vi "Voir alertes.vi"() -> ()   [LabVIEW 2022 SP3]
uses:
  Enum/Enum 8.ctl
  Variables globales/Variable glob alertes ecart temperatures.vi
  Variables globales/Variable glob alertes pressions.vi
  Variables globales/Variable glob alertes min-max temperatures.vi
  Variables globales/Variable glob mails.vi
  Variables globales/Variable glob alertes Compteurs.vi
  Variables globales/Variable glob alertes Keller.vi
panel:
  out "référence en sortie":refnum<vi>
  in  "stop":bool
  in  "Commande onglets":T1(tab)
  out "min-max temp":T2(array[cluster]) {"alerte min (°C) :" format="%.2f"; "alerte max (°C) :" format="%.2f"}
  out "écarts températures":T3(array[cluster]) {"alerte écart (°C) :" format="%.2f"}
  out "Pressions":T4(array[cluster]) {"alerte pression (mbar) :" format="%.2e"}
  out "Keller":T5(array[cluster]) {"alerte keller (mbar) :" format="%.2g"}
  out "Copmteurs":T6(array[cluster]) {"alerte débit compteurs (m3/h) :" format="%.2g"}
  out "Liste mails envoi alertes":string[](array[string])
  # "capteurs surveillés :"
  # "Ce logiciel et les informations qu'il contient, sont la propriété de l’IAS \net ne peuvent être diffusés sans l’autorisation de la Station d’étalonnage"
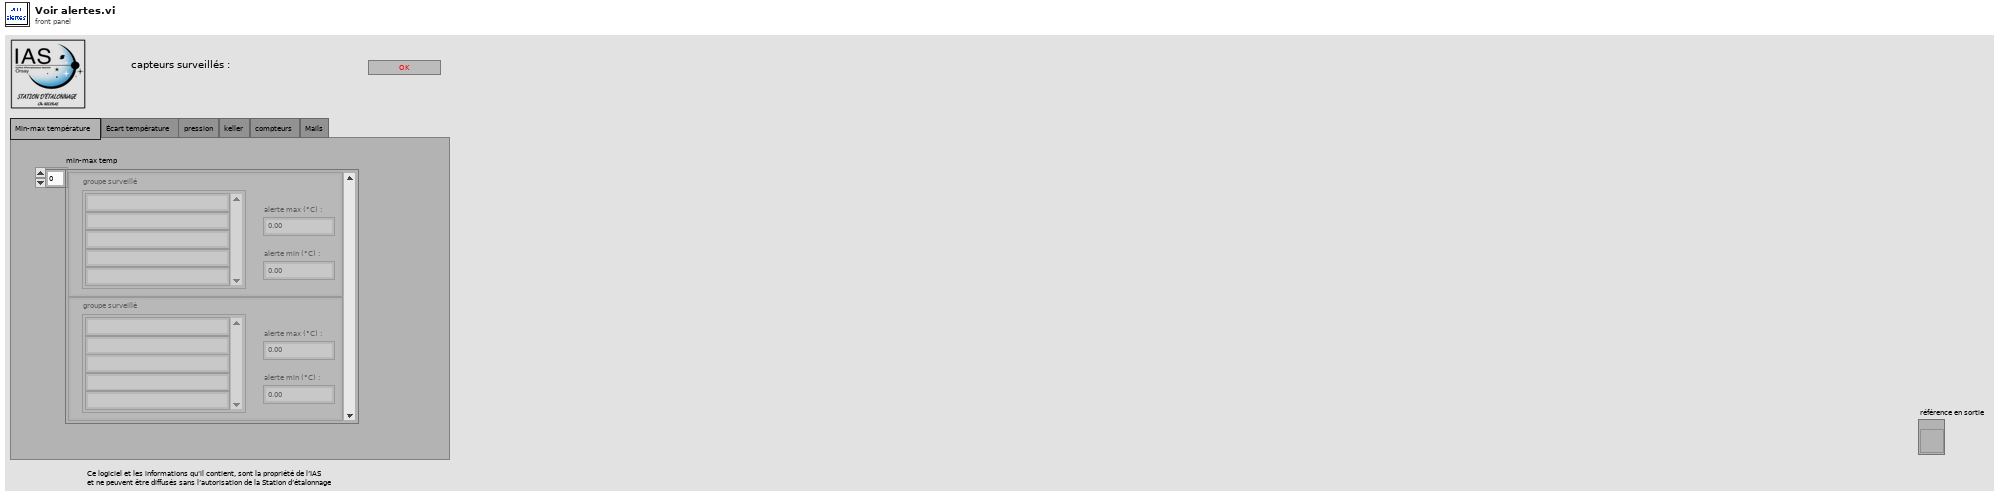
[diagram p1: front panel]
types:
  T1 = enum32{"Min-max température", "Écart température", "pression", "keller", "compteurs", "Mails"}
  T2 = cluster{"groupe surveillé":string[], "alerte max (°C) :":dbl, "alerte min (°C) :":dbl}[]
  T3 = cluster{"capteurs temp surveillés":string[], "alerte écart (°C) :":dbl, ">?":bool}[]
  T4 = cluster{"capteurs pression surveillés":string[], "alerte pression (mbar) :":dbl}[]
  T5 = cluster{"capteurs keller surveillés":string[], "alerte keller (mbar) :":dbl}[]
  T6 = cluster{"compteurs débit surveillés":string[], "alerte débit compteurs (m3/h) :":dbl}[]
  T7 = typedef "Enum 8.ctl" = enum16{"init", "variables", "variables 2", "onglets", "attente", "fin"}
  T8 = enum32{"Invalid", "Standard", "Closed", "Hidden", "Minimized", "Maximized"}
  T9 = cluster{"Alerte temp min/max":bool, "température max":dbl, "température min":dbl, "Défaut min/max temp":bool, "Indices à controler":i16[], "N°":u16}[]
  T10 = cluster{"Indices a controler":i16[], "Defaut":bool, "ecart temp":dbl, "Alerte":bool, ">?":bool, "N°":u16}[]
  T11 = cluster{"Alerte":bool, "valeur ":dbl, "Défaut":bool, "Indices controler":i16[], "N°":u16}[]
  T12 = cluster{"capteurs temp surveillés":string[], "alerte écart (°C) :":dbl, ">?":bool}
  T13 = cluster{"capteurs pression surveillés":string[], "alerte pression (mbar) :":dbl}
  T14 = cluster{"groupe surveillé":string[], "alerte max (°C) :":dbl, "alerte min (°C) :":dbl}
  T15 = cluster{"Alerte":bool, "valeur alerte":dbl, "Défaut":bool, "Indices à controler":i16[], "N°":u16}[]
  T16 = cluster{"Alerte Keller":bool, "valeur alerte Keller":dbl, "Défaut Keller":bool, "Indices Keller à controler":i16[], "N°":u16}[]
  T17 = cluster{"compteurs débit surveillés":string[], "alerte débit compteurs (m3/h) :":dbl}
  T18 = cluster{"capteurs keller surveillés":string[], "alerte keller (mbar) :":dbl}
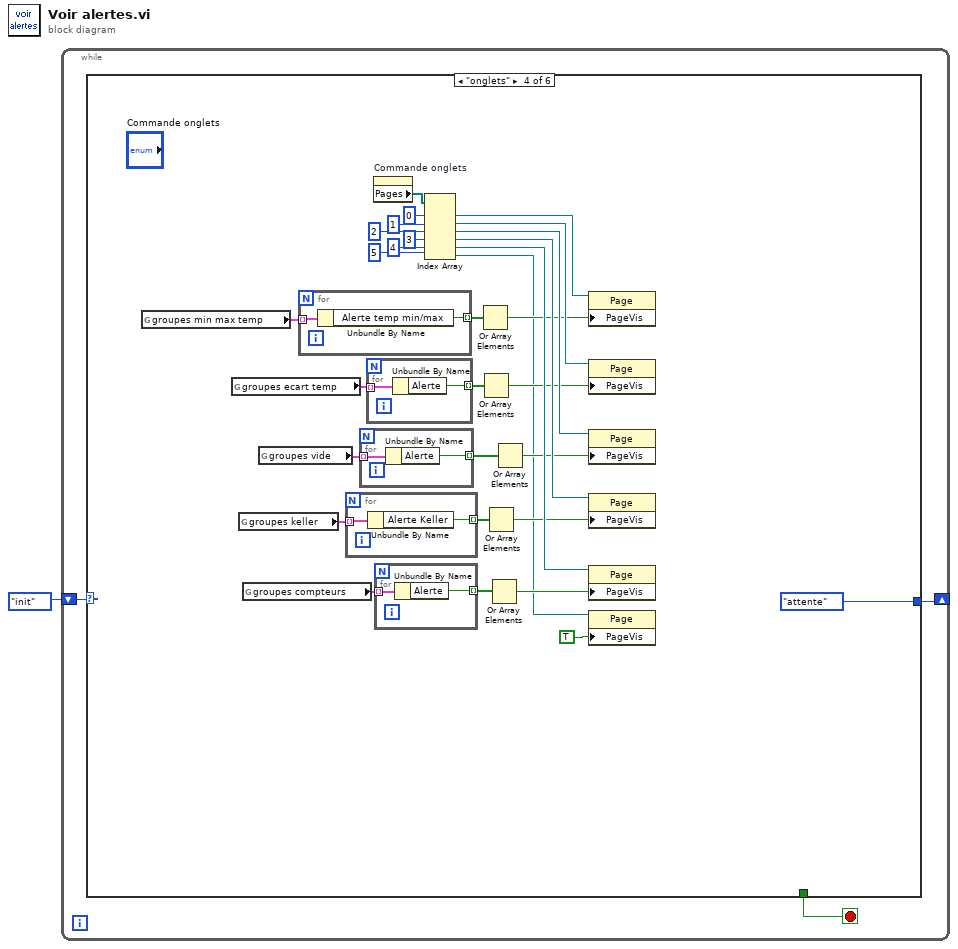
[diagram p0: block diagram]
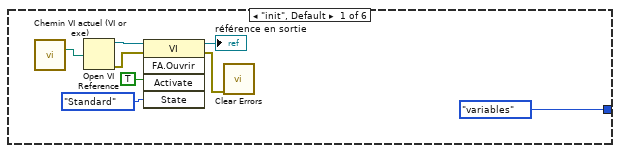
[diagram p2: hidden frame]
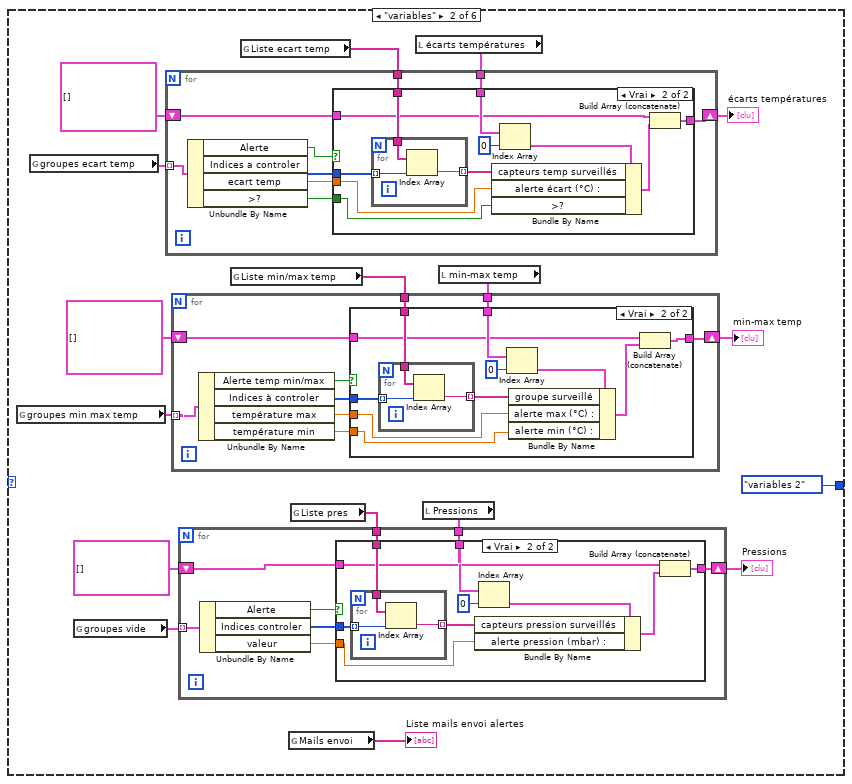
[diagram p3: hidden frame]
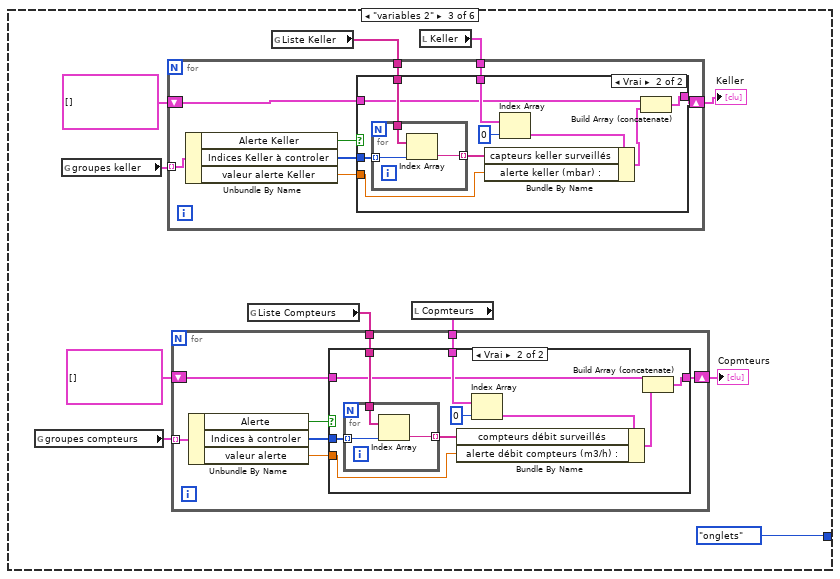
[diagram p7: hidden frame]
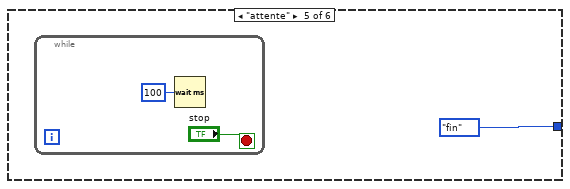
[diagram p10: hidden frame]
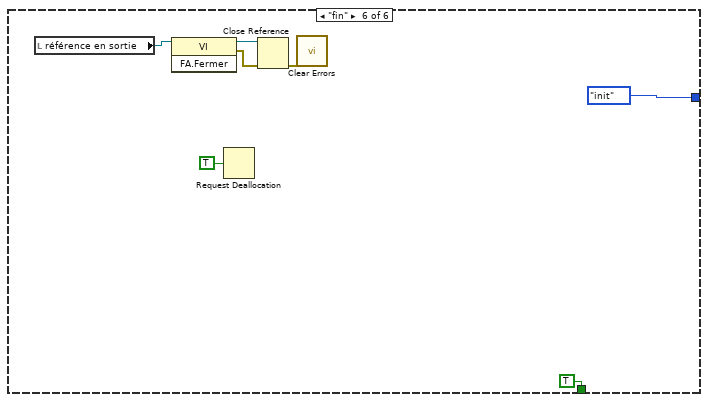
[diagram p11: hidden frame]
diagram:
  n1 = while {
    shift-right: [w3] -> _
    shift-left: Enum_8."init" ("Énum") -> [w4]
    stop <- w2 stop-if-true
    n2 = case shown="\"onglets\"" w4 {
      tunnel: [Enum_8."variables" ("Énum") Enum_8."variables 2" ("Énum") Enum_8."onglets" ("Énum") Enum_8."attente" ("Énum") Enum_8."fin" ("Énum") Enum_8."init" ("Énum")] -> w3
      tunnel: [_ _ _ _ _ TRUE] -> w2
      frame "init", Default {
        n3 = call "Chemin VI actuel (VI or exe).vi"() -> ("Full Path to VI or executable"=w5:path)  [unwired: 14 in, 1 out]
        n4 = Open VI Reference(vi path=w5) -> (vi reference=w9:refnum<vi>, error out=w11:errorcluster)  [unwired: 5 in]
        n5 = invoke class="VI" method="FA.Ouvrir"(reference=w9, error in=w11, "Activate"=TRUE ("Activer ?"), "State"=T8."Standard" ("État")) -> (reference out=→"référence en sortie":refnum<vi>, error out=w12:errorcluster)  [unwired: 1 in, 3 out]
        n6 = call <vilib>:"Clear Errors.vi"("error in (no error)"=w12) -> ()  [unwired: 5 in, 2 out]
      }
      frame "variables" {
        n7 = global read "Variable glob alertes min-max temperatures.vi" "groupes min max temp"() -> (w24:T9)
        n8 = global read "Variable glob alertes ecart temperatures.vi" "groupes ecart temp"() -> (w28:T10)
        n9 = global read "Variable glob alertes pressions.vi" "groupes vide"() -> (w21:T11)
        n10 = global read "Variable glob alertes min-max temperatures.vi" "Liste min/max temp"() -> (w23:string[])
        n11 = global read "Variable glob alertes ecart temperatures.vi" "Liste ecart temp"() -> (w27:string[])
        n12 = global read "Variable glob mails.vi" "Mails envoi"() -> (→"Liste mails envoi alertes":string[])
        n13 = global read "Variable glob alertes pressions.vi" "Liste pres"() -> (w22:string[])
        n14 = local read "écarts températures"() -> (w26:T3)
        n15 = for {
          tunnel: w28 -> [w84] mode=indexing
          tunnel: w27 -> [w82]
          tunnel: w26 -> [w81]
          shift-right: [w76] -> w20
          shift-left: T3 [] -> [w77]
          n16 = Unbundle By Name(w84) -> ("Alerte"=w79:bool, "Indices a controler"=w83:i16[], "ecart temp"=w80:dbl, ">?"=w78:bool)
          n17 = case shown="Vrai" w79 {
            tunnel: w83 -> [_ w96]
            tunnel: w82 -> [_ w95]
            tunnel: w81 -> [_ w94]
            tunnel: w80 -> [_ w90]
            tunnel: w78 -> [_ w89]
            tunnel: w77 -> [w85 w87]
            tunnel: [w85 w86] -> w76
            frame False {
            }
            frame True {
              n18 = for {
                tunnel: w96 -> [w98] mode=indexing
                tunnel: w95 -> [w99]
                tunnel: [w97] -> w91 mode=indexing
                n19 = Index Array(array=w99, index=w98) -> (element=w97:string)
              }
              n20 = Index Array(array=w94, index=0 ("indice")) -> (element=w92:T12)
              n21 = Bundle By Name(cluster=w92, "capteurs temp surveillés"=w91, "alerte écart (°C) :"=w90, ">?"=w89) -> (w88:T12)
              n22 = Build Array (concatenate)(w87, w88) -> (w86:T3)
            }
          }
        }
        "écarts températures" <- w20
        n23 = local read "Pressions"() -> (w16:T4)
        n24 = for {
          tunnel: w21 -> [w37] mode=indexing
          tunnel: w22 -> [w35]
          tunnel: w16 -> [w34]
          shift-right: [w30] -> w15
          shift-left: T4 [] -> [w31]
          n25 = Unbundle By Name(w37) -> ("Alerte"=w32:bool, "Indices controler"=w36:i16[], "valeur"=w33:dbl)
          n26 = case shown="Vrai" w32 {
            tunnel: w36 -> [_ w48]
            tunnel: w35 -> [_ w47]
            tunnel: w34 -> [_ w46]
            tunnel: w33 -> [_ w42]
            tunnel: w31 -> [w38 w40]
            tunnel: [w38 w39] -> w30
            frame False {
            }
            frame True {
              n27 = for {
                tunnel: w48 -> [w50] mode=indexing
                tunnel: w47 -> [w51]
                tunnel: [w49] -> w43 mode=indexing
                n28 = Index Array(array=w51, index=w50) -> (element=w49:string)
              }
              n29 = Index Array(array=w46, index=0 ("indice")) -> (element=w44:T13)
              n30 = Bundle By Name(cluster=w44, "capteurs pression surveillés"=w43, "alerte pression (mbar) :"=w42) -> (w41:T13)
              n31 = Build Array (concatenate)(w40, w41) -> (w39:T4)
            }
          }
        }
        "Pressions" <- w15
        n32 = local read "min-max temp"() -> (w25:T2)
        n33 = for {
          tunnel: w24 -> [w60] mode=indexing
          tunnel: w23 -> [w58]
          tunnel: w25 -> [w57]
          shift-right: [w52] -> w17
          shift-left: T2 [] -> [w53]
          n34 = Unbundle By Name(w60) -> ("Alerte temp min/max"=w54:bool, "Indices à controler"=w59:i16[], "température max"=w56:dbl, "température min"=w55:dbl)
          n35 = case shown="Vrai" w54 {
            tunnel: w59 -> [_ w72]
            tunnel: w58 -> [_ w71]
            tunnel: w57 -> [_ w70]
            tunnel: w56 -> [_ w66]
            tunnel: w55 -> [_ w65]
            tunnel: w53 -> [w61 w63]
            tunnel: [w61 w62] -> w52
            frame False {
            }
            frame True {
              n36 = for {
                tunnel: w72 -> [w74] mode=indexing
                tunnel: w71 -> [w75]
                tunnel: [w73] -> w67 mode=indexing
                n37 = Index Array(array=w75, index=w74) -> (element=w73:string)
              }
              n38 = Index Array(array=w70, index=0 ("indice")) -> (element=w68:T14)
              n39 = Bundle By Name(cluster=w68, "groupe surveillé"=w67, "alerte max (°C) :"=w66, "alerte min (°C) :"=w65) -> (w64:T14)
              n40 = Build Array (concatenate)(w63, w64) -> (w62:T2)
            }
          }
        }
        "min-max temp" <- w17
      }
      frame "variables 2" {
        n41 = global read "Variable glob alertes Compteurs.vi" "groupes compteurs"() -> (w103:T15)
        n42 = global read "Variable glob alertes Keller.vi" "groupes keller"() -> (w105:T16)
        n43 = global read "Variable glob alertes Compteurs.vi" "Liste Compteurs"() -> (w104:string[])
        n44 = global read "Variable glob alertes Keller.vi" "Liste Keller"() -> (w107:string[])
        n45 = local read "Copmteurs"() -> (w102:T6)
        n46 = for {
          tunnel: w103 -> [w118] mode=indexing
          tunnel: w104 -> [w116]
          tunnel: w102 -> [w115]
          shift-right: [w111] -> w109
          shift-left: T6 [] -> [w112]
          n47 = Unbundle By Name(w118) -> ("Alerte"=w113:bool, "Indices à controler"=w117:i16[], "valeur alerte"=w114:dbl)
          n48 = case shown="Vrai" w113 {
            tunnel: w117 -> [_ w129]
            tunnel: w116 -> [_ w128]
            tunnel: w115 -> [_ w127]
            tunnel: w114 -> [_ w123]
            tunnel: w112 -> [w119 w121]
            tunnel: [w119 w120] -> w111
            frame False {
            }
            frame True {
              n49 = for {
                tunnel: w129 -> [w131] mode=indexing
                tunnel: w128 -> [w132]
                tunnel: [w130] -> w124 mode=indexing
                n50 = Index Array(array=w132, index=w131) -> (element=w130:string)
              }
              n51 = Index Array(array=w127, index=0 ("indice")) -> (element=w125:T17)
              n52 = Bundle By Name(cluster=w125, "compteurs débit surveillés"=w124, "alerte débit compteurs (m3/h) :"=w123) -> (w122:T17)
              n53 = Build Array (concatenate)(w121, w122) -> (w120:T6)
            }
          }
        }
        "Copmteurs" <- w109
        n54 = local read "Keller"() -> (w106:T5)
        n55 = for {
          tunnel: w105 -> [w140] mode=indexing
          tunnel: w107 -> [w138]
          tunnel: w106 -> [w137]
          shift-right: [w133] -> w108
          shift-left: T5 [] -> [w134]
          n56 = Unbundle By Name(w140) -> ("Alerte Keller"=w135:bool, "Indices Keller à controler"=w139:i16[], "valeur alerte Keller"=w136:dbl)
          n57 = case shown="Vrai" w135 {
            tunnel: w139 -> [_ w151]
            tunnel: w138 -> [_ w150]
            tunnel: w137 -> [_ w149]
            tunnel: w136 -> [_ w145]
            tunnel: w134 -> [w141 w143]
            tunnel: [w141 w142] -> w133
            frame False {
            }
            frame True {
              n58 = for {
                tunnel: w151 -> [w153] mode=indexing
                tunnel: w150 -> [w154]
                tunnel: [w152] -> w146 mode=indexing
                n59 = Index Array(array=w154, index=w153) -> (element=w152:string)
              }
              n60 = Index Array(array=w149, index=0 ("indice")) -> (element=w147:T18)
              n61 = Bundle By Name(cluster=w147, "capteurs keller surveillés"=w146, "alerte keller (mbar) :"=w145) -> (w144:T18)
              n62 = Build Array (concatenate)(w143, w144) -> (w142:T5)
            }
          }
        }
        "Keller" <- w108
      }
      frame "onglets" {
        n63 = global read "Variable glob alertes min-max temperatures.vi" "groupes min max temp"() -> (w170:T9)
        n64 = global read "Variable glob alertes ecart temperatures.vi" "groupes ecart temp"() -> (w166:T10)
        n65 = global read "Variable glob alertes Keller.vi" "groupes keller"() -> (w163:T16)
        n66 = global read "Variable glob alertes Compteurs.vi" "groupes compteurs"() -> (w158:T15)
        n67 = global read "Variable glob alertes pressions.vi" "groupes vide"() -> (w161:T11)
        n68 = for {
          tunnel: w170 -> [w194] mode=indexing
          tunnel: [w193] -> w169 mode=indexing
          n69 = Unbundle By Name(w194) -> ("Alerte temp min/max"=w193:bool)
        }
        n70 = for {
          tunnel: w163 -> [w190] mode=indexing
          tunnel: [w189] -> w164 mode=indexing
          n71 = Unbundle By Name(w190) -> ("Alerte Keller"=w189:bool)
        }
        n72 = for {
          tunnel: w161 -> [w188] mode=indexing
          tunnel: [w187] -> w160 mode=indexing
          n73 = Unbundle By Name(w188) -> ("Alerte"=w187:bool)
        }
        n74 = for {
          tunnel: w166 -> [w192] mode=indexing
          tunnel: [w191] -> w167 mode=indexing
          n75 = Unbundle By Name(w192) -> ("Alerte"=w191:bool)
        }
        n76 = property on="Commande onglets" class="Onglet (strict)"() -> ("Pages"=w184:refnum<vi>[])  [unwired: 2 in, 2 out]
        n77 = for {
          tunnel: w158 -> [w186] mode=indexing
          tunnel: [w185] -> w157 mode=indexing
          n78 = Unbundle By Name(w186) -> ("Alerte"=w185:bool)
        }
        n79 = Index Array(array=w184, index #1=0 ("indice"), index #2=1 ("indice"), index #3=2 ("indice"), index #4=3 ("indice"), index #5=4 ("indice"), index #6=5 ("indice")) -> (element #1=w179:refnum<vi>, element #2=w180:refnum<vi>, element #3=w181:refnum<vi>, element #4=w182:refnum<vi>, element #5=w183:refnum<vi>, element #6=w155:refnum<vi>)
        n80 = Or Array Elements(Boolean array=w169) -> (logical OR=w168:bool)
        n81 = Or Array Elements(Boolean array=w167) -> (logical OR=w165:bool)
        n82 = Or Array Elements(Boolean array=w164) -> (logical OR=w162:bool)
        n83 = Or Array Elements(Boolean array=w157) -> (logical OR=w156:bool)
        n84 = Or Array Elements(Boolean array=w160) -> (logical OR=w159:bool)
        n85 = property class="Page"(reference=w179, "PageVis"=w168) -> ()  [unwired: 1 in, 2 out]
        n86 = property class="Page"(reference=w180, "PageVis"=w165) -> ()  [unwired: 1 in, 2 out]
        n87 = property class="Page"(reference=w181, "PageVis"=w159) -> ()  [unwired: 1 in, 2 out]
        n88 = property class="Page"(reference=w182, "PageVis"=w162) -> ()  [unwired: 1 in, 2 out]
        n89 = property class="Page"(reference=w183, "PageVis"=w156) -> ()  [unwired: 1 in, 2 out]
        n90 = property class="Page"(reference=w155, "PageVis"=TRUE ("Page visible")) -> ()  [unwired: 1 in, 2 out]
      }
      frame "attente" {
        n91 = while {
          stop <- "stop" stop-if-true
          n92 = Wait (ms)(milliseconds to wait=u32 100 ("attente (ms)")) -> ()  [unwired: 1 out]
        }
      }
      frame "fin" {
        n93 = local read "référence en sortie"() -> (w200:refnum<vi>)
        n94 = invoke class="VI" method="FA.Fermer"(reference=w200) -> (reference out=w202:refnum<vi>, error out=w201:errorcluster)  [unwired: 2 in, 1 out]
        n95 = Request Deallocation(TRUE ("flag")) -> ()
        n96 = Close Reference(reference=w202, error in (no error)=w201) -> (error out=w203:errorcluster)
        n97 = call <vilib>:"Clear Errors.vi"("error in (no error)"=w203) -> ()  [unwired: 5 in, 2 out]
      }
    }
  }
